vi "MoveForwards.vi"(0 "Time On (100ms)":dbl=1.0, 1 "NXT/EV3 IN":T2, 2 "Motor IDs":cluster{"Motors":T1, "Motors 2":T1}={"Motors"=0, "Motors 2"=1} {"Motors 2" items=["Port A", "Port B", "Port C", "Port D"]; "Motors" items=["Port A", "Port B", "Port C", "Port D"]}, 3 "Power":dbl) -> (4 "NXT/EV3 OUT":T2)   [LabVIEW 2016, in "13.03 Robot.lvrbt"]
uses:
  13.03 Robot.lvrbt
  <vilib>/NXT/Subs/LVHSConnector.ctl
  <vilib>/NXT/LegoClasses/BrickReference/BrickReference.lvclass
  <vilib>/NXT/Block Support/NXT_OutputPort.ctl
  <vilib>/NXT/NXTIO Xnodes/NXTIONodeSubVIs/NXTMoveMotors.vi
  <vilib>/NXT/NXTIO Xnodes/NXTIOXNode/NXTIO.xnode
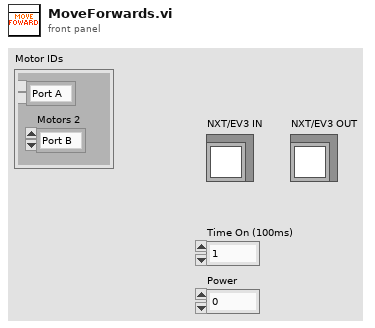
[diagram p1: front panel]
types:
  T1 = typedef "NXT_OutputPort.ctl" = u8
  T2 = typedef "LVHSConnector.ctl" = refnum<class "BrickReference.lvclass">
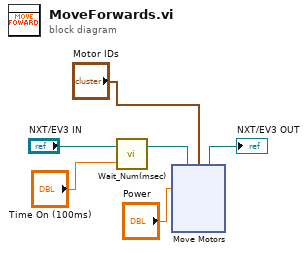
[diagram p0: block diagram]
diagram:
  n1 = call <vilib>:"Wait_Num(msec).vi"("Time (100 msec)"="Time On (100ms)", "NXT/EV3"="NXT/EV3 IN") -> ("NXT/EV3"=w6:T2)  [unwired: 2 in]
  n2 = xnode "Move Motors"("Power/Speed 2"="Power", "Power/Speed 1"="Power", "Motors"="Motor IDs", "NXT/EV3"=w6) -> ("NXT/EV3"=→"NXT/EV3 OUT":T2)
